vi "Hash Whitelist--constant.vi"() -> (2 "Hash Values":string[](array[string]), 3 "Files":string[](array[string]))   [LabVIEW 2026]
doc: "This constant represent hash values of file that are allowed to be run. This actual values must be filled during project creation automatically so that they are baked into the built ppl (and thus not modifiable for the end user)."
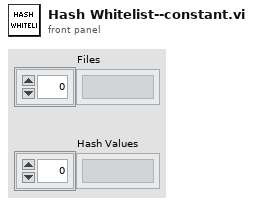
[diagram p1: front panel]
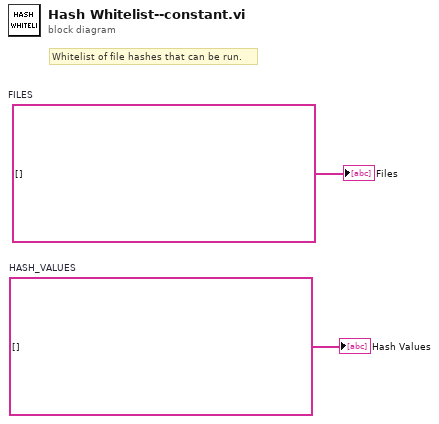
[diagram p0: block diagram]
diagram:
  w1 = string[] []  # HASH_VALUES
  w2 = string[] []  # FILES
  # "Whitelist of file hashes that can be run."
  "Files" <- w2
  "Hash Values" <- w1
